vi "List Phone Numbers Recursive.vi"(8 "error in (no error)":errorcluster, 10 "nextToken":string, 11 "Phone Number":refnum<class "Phone Number.lvclass">) -> (0 "error out":errorcluster, 3 "Phone Numbers Opted Out":refnum<class "Phone Number.lvclass">[](array[class]))   [LabVIEW 2015, in "NI_AWS_SNS.lvlib" / "Phone Number.lvclass"]
uses:
  Phone Number.lvclass
  Core/HTTP Request/Request Options.ctl
  Core/HTTP Request/Name Value Pair.ctl
  Core/HTTP Request/Region handling.ctl
  Core/HTTP Request/URL formatting.ctl
  Phone Number.lvclass/Phone Number.ctl
  Write Phone Number.vi
  Core/HTTP Request/HTTP Request.lvclass
  XML Parsing/NI_XML Parsing.lvlib
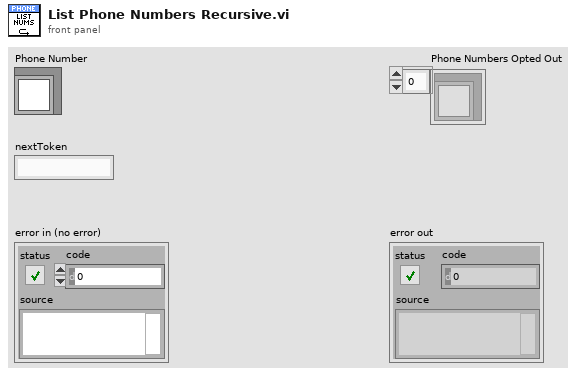
[diagram p1: front panel]
types:
  T1 = typedef "NI_AWS_Core.lvlib/HTTP Request.lvclass/Name Value Pair.ctl" = cluster{"name":string, "value":string}
  T2 = typedef "NI_AWS_Core.lvlib/HTTP Request.lvclass/Request Options.ctl" = cluster{"request headers":T1[], "request parameters":T1[], "request body":string, "region handling":T3, "URL formatting":T4}
  T3 = typedef "NI_AWS_Core.lvlib/HTTP Request.lvclass/Region handling.ctl" = enum16{"use region everywhere", "use region (authentication only)", "use region (URL only)", "ignore region everwhere"}
  T4 = typedef "NI_AWS_Core.lvlib/HTTP Request.lvclass/URL formatting.ctl" = enum16{"region-", "region."}
  T5 = typedef "NI_AWS_Core.lvlib/HTTP Request.lvclass/Response.ctl" = cluster{"Headers":string, "Body":string}
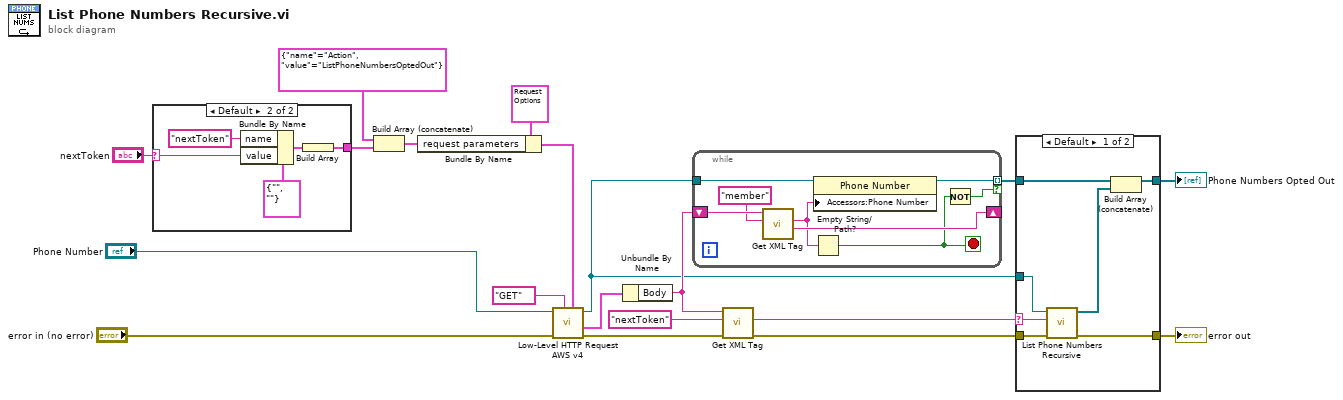
[diagram p0: block diagram]
diagram:
  n1 = case shown="Default" "nextToken" {
    selector: "nextToken" -> [_ w24]
    tunnel: [_ w20] -> w18
    frame "" {
    }
    frame Default {
      n2 = Bundle By Name(cluster=T1 {"name"="", "value"=""} ("Name Value Pair"), "name"="nextToken", "value"=w24) -> (w22:T1)
      n3 = Build Array(w22) -> (w20:T1[])
    }
  }
  n4 = Build Array (concatenate)(T1 {"name"="Action", "value"="ListPhoneNumbersOptedOut"} ("Name Value Pair"), w18) -> (w16:T1[])
  n5 = Bundle By Name(cluster=T2 {"request headers"=[], "request parameters"=[{"name"="Action", "value"="ListQueues"}], "request body"="", "region handling"=enum."use region everywhere", "URL formatting"=enum."region."} ("Request Options"), "request parameters"=w16) -> (w1:T2)
  n6 = call "Low-Level HTTP Request AWS v4.vi"("Request Options"=w1, "HTTP-Verb"="GET", "error in (no error)"="error in (no error)", "AWS Core in"="Phone Number") -> ("error out"=w7:errorcluster, "Response"=w5:T5, "AWS Core out"=w2:refnum<class "Phone Number.lvclass">)  [unwired: 4 in, 1 out]
  n7 = Unbundle By Name(w5) -> ("Body"=w13:string)
  n8 = while {
    shift-right: [w30] -> _
    shift-left: w13 -> [w32]
    tunnel: w2 -> [w29]
    tunnel: [w28] -> w10 mode=indexing if=w26
    stop <- w25 stop-if-true
    n9 = call "Get XML Tag.vi"("Tag name"="member", "XML String in"=w32) -> ("Remaining string"=w30:string, "Tag value"=w27:string)  [unwired: 5 in, 3 out]
    n10 = Empty String/Path?(string/path=w27) -> (empty?=w25:bool)
    n11 = property class="Phone Number"(reference=w29, "Accessors:Phone Number"=w27) -> (reference out=w28:refnum<class "Phone Number.lvclass">)  [unwired: 1 in, 1 out]
    n12 = Not(x=w25) -> (.not. x?=w26:bool)
  }
  n13 = call "Get XML Tag.vi"("error in (no error)"=w7, "Tag name"="nextToken", "XML String in"=w13) -> ("error out"=w6:errorcluster, "Tag value"=w11:string)  [unwired: 4 in, 3 out]
  n14 = case shown="Default" w11 {
    selector: w11 -> [w38 _]
    tunnel: w10 -> [w37 w41]
    tunnel: [w36 w41] -> w9
    tunnel: w6 -> [w39 w40]
    tunnel: [w35 w40] -> w8
    tunnel: w2 -> [w33 _]
    frame Default {
      n15 = call "List Phone Numbers Recursive.vi"("error in (no error)"=w39, "nextToken"=w38, "Phone Number"=w33) -> ("error out"=w35:errorcluster, "Phone Numbers Opted Out"=w34:refnum<class "Phone Number.lvclass">[])  [unwired: 7 in]
      n16 = Build Array (concatenate)(w37, w34) -> (w36:refnum<class "Phone Number.lvclass">[])
    }
    frame "" {
    }
  }
  "error out" <- w8
  "Phone Numbers Opted Out" <- w9
